vi "pluto_acquisition_test.vi"() -> ()   [LabVIEW 2026]
uses:
  <vilib>/Analysis/baseanly.llb/Mean (DBL).vi
  <vilib>/Python/Open Venv Python Session.vi
  <vilib>/Analysis/NI_AALBase.lvlib
panel:
  out "RMS Magnitude":dbl
  out "Mean I/Q Power":dbl format="%0.2f"
  out "Q Array Length":i32
  out "I Array Length":i32
  out "return value":cluster{bool, dbl[], dbl[], i32, string}
  out "error out":errorcluster
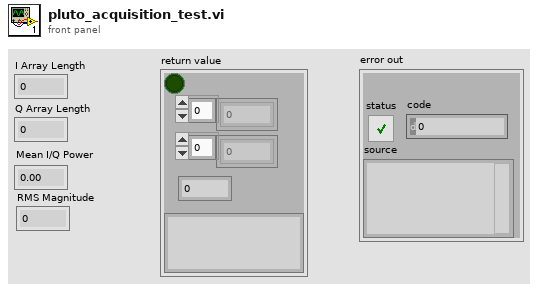
[diagram p1: front panel]
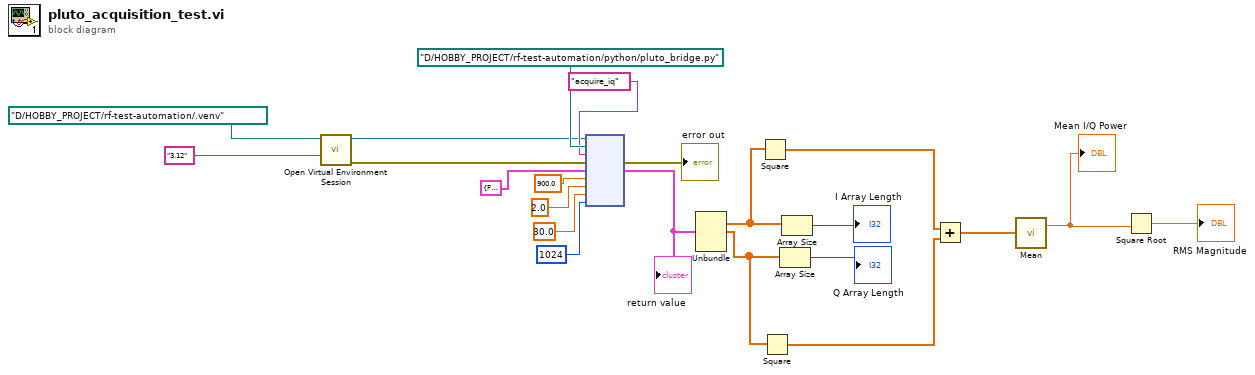
[diagram p0: block diagram]
diagram:
  n1 = call-poly <vilib>:"Open Virtual Environment Session.vi"("Python version"="3.12", "Env path"=path "D:/HOBBY_PROJECT/rf-test-automation/.venv") -> ("error out"=w19:errorcluster, "session out"=w20:refnum<k35>)  [unwired: 8 in]
  n2 = node(w20, path "D:/HOBBY_PROJECT/rf-test-automation/python/pluto_bridge.py" ("module path"), "acquire_iq" ("function name"), w19, cluster{bool, dbl[], dbl[], i32, string} {FALSE, [], [], 0, ""}, 900.0, 2.0, 30.0, 1024) -> (→"error out":errorcluster, w10:cluster{bool, dbl[], dbl[], i32, string})  [unwired: 4 in, 3 out]
  "return value" <- w10
  n3 = Unbundle(w10) -> (w7:dbl[], w6:dbl[])  [unwired: 3 out]
  n4 = Square(x=w7) -> (x^2=w5:dbl[])
  n5 = Square(x=w6) -> (x^2=w4:dbl[])
  n6 = Array Size(array=w6) -> (size(s)=→"Q Array Length":i32)
  n7 = Array Size(array=w7) -> (size(s)=→"I Array Length":i32)
  n8 = Add(x=w5, y=w4) -> (x+y=w3:dbl[])
  n9 = call-poly <vilib>:"Mean.vi"("X"=w3) -> ("mean"=w2:dbl)  [unwired: 1 out]
  "Mean I/Q Power" <- w2
  n10 = Square Root(x=w2) -> (sqrt(x)=→"RMS Magnitude":dbl)
